vi "Module Loop.vi"(8 "error in (no error)":errorcluster, 11 "Telemetry Server Module in":refnum<class "Telemetry Server Module.lvclass">) -> (0 "error out":errorcluster, 3 "Telemetry Server Module out":refnum<class "Telemetry Server Module.lvclass">)   [LabVIEW 2020, in "Volatus.lvlib" / "Telemetry Server Module.lvclass"]
uses:
  Telemetry Server Module.lvclass
  Telemetry Server Module.lvclass/Telemetry Server Module.ctl
  Module/Module.lvclass
  C:/dev/lv20CE/relink/lv-volatus/Volatus/Module/Module.lvclass
  C:/dev/lv20CE/relink/lv-volatus/Volatus/Telemetry Server Module/Telemetry Server Module.lvclass
  lv-vecto/Vecto/IP Resolver/IP Resolver.lvclass
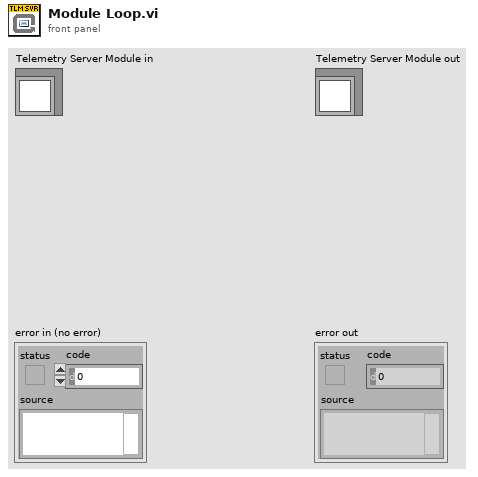
[diagram p1: front panel]
types:
  T1 = enum32{"Invalid", "Standard", "Closed", "Hidden", "Minimized", "Maximized"}
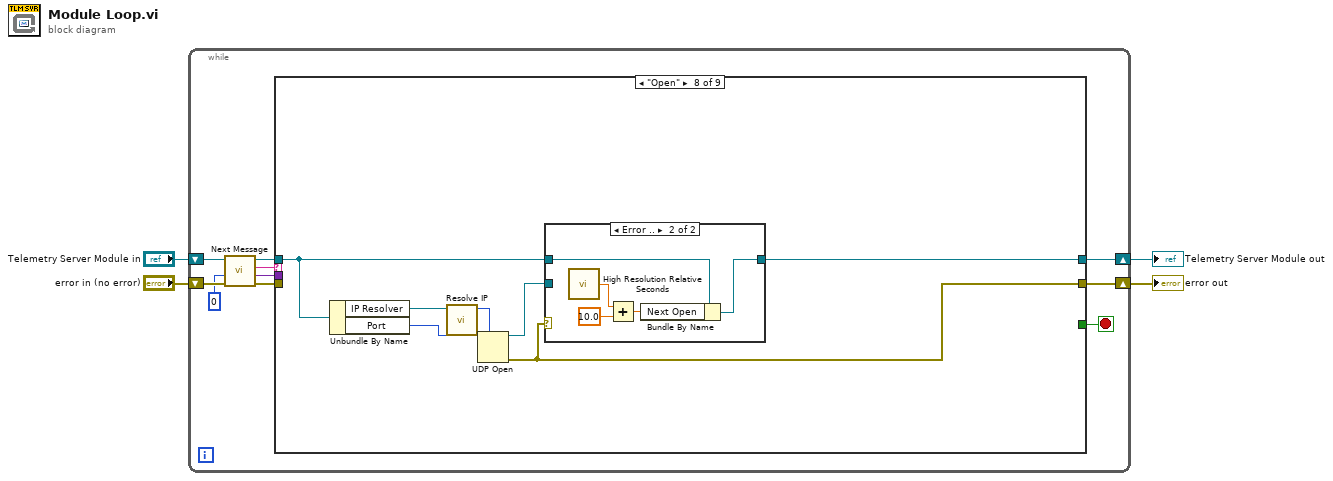
[diagram p0: block diagram]
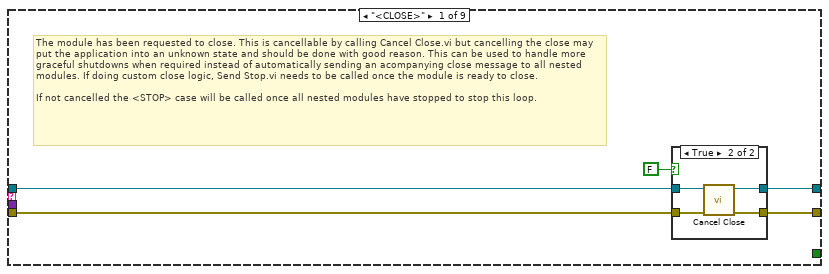
[diagram p2: hidden frame]
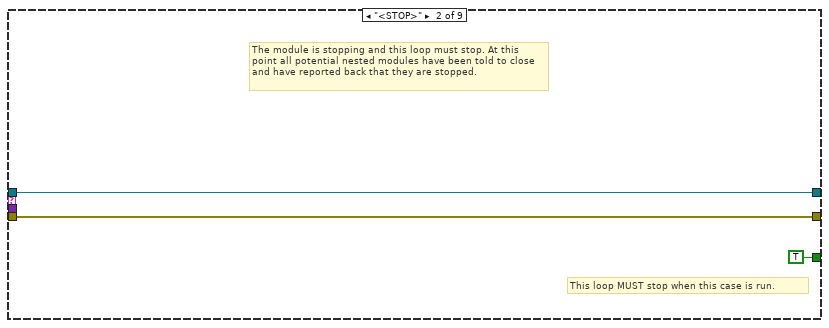
[diagram p4: hidden frame]
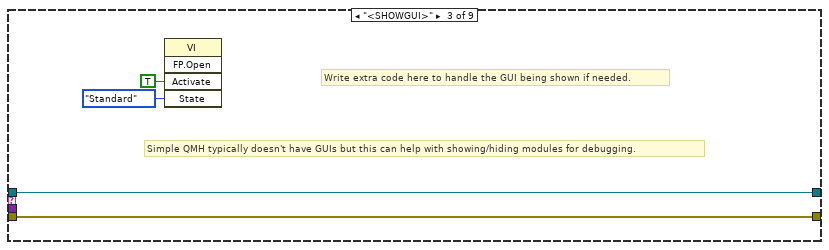
[diagram p5: hidden frame]
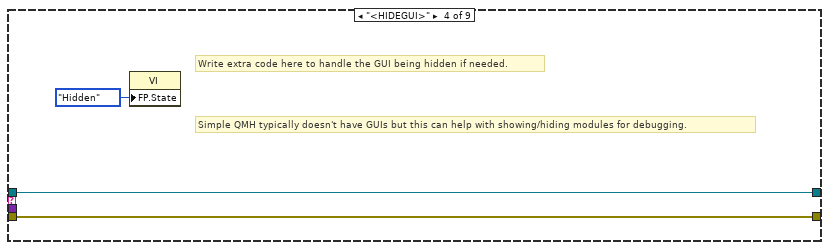
[diagram p6: hidden frame]
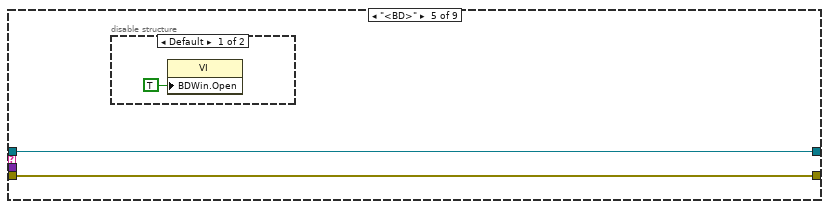
[diagram p7: hidden frame]
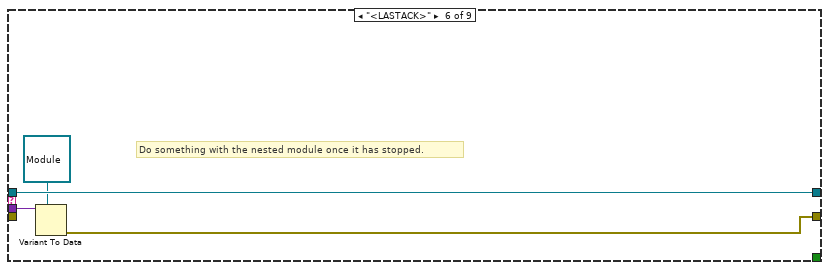
[diagram p9: hidden frame]
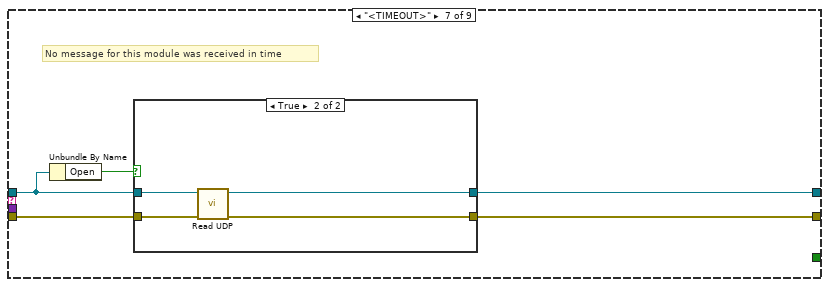
[diagram p10: hidden frame]
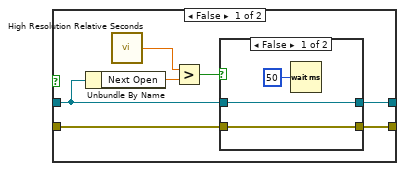
[diagram p11: hidden frame]
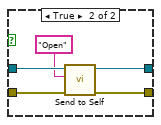
[diagram p12: hidden frame]
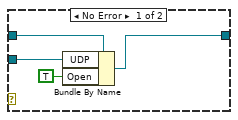
[diagram p13: hidden frame]
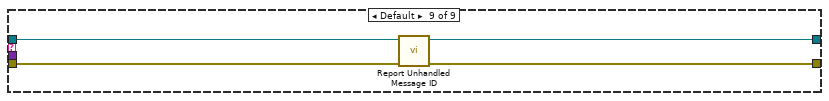
[diagram p14: hidden frame]
diagram:
  n1 = while {
    shift-right: [w9] -> w2
    shift-left: "Telemetry Server Module in" -> [w14]
    shift-right: [w8] -> w1
    shift-left: "error in (no error)" -> [w13]
    stop <- w7 stop-if-true
    n2 = call "Next Message.vi"("error in (no error)"=w13, "Timeout ms (-1)"=0, "Module in"=w14) -> ("error out"=w12:errorcluster, "Data"=w6:variant, "ID"=w11:string, "Module out"=w10:refnum<class "Telemetry Server Module.lvclass">)  [unwired: 5 in]
    n3 = case shown="\"Open\"" w11 {
      tunnel: w12 -> [w19 w27 w31 w34 w36 _ w47 _ w86]
      tunnel: w10 -> [w17 w28 w32 w35 w37 w42 w44 w73 w84]
      tunnel: [w16 w28 w32 w35 w37 w42 w45 w69 w83] -> w9
      tunnel: [w18 w27 w31 w34 w36 w39 w46 w67 w85] -> w8
      tunnel: [_ TRUE _ _ _ _ _ _ _] -> w7
      tunnel: w6 -> [_ _ _ _ _ w41 _ _ _]
      frame "<CLOSE>" {
        # "The module has been requested to close. This is cancellable by calling Cancel Close.vi but cancelling the close may put the application into an unknown state and should be done with good reason. This can be used to handle more graceful shutdowns when required instead of automatically sending an acompanying close message to all nested modules. If doing custom close logic, Send Stop.vi needs to be called once the module is ready to close.\n\nIf not cancelled the <STOP> case will be called once all nested modules have stopped to stop this loop."
        n4 = case shown="True" FALSE {
          tunnel: w19 -> [w20 w25]
          tunnel: [w20 w24] -> w18
          tunnel: w17 -> [w21 w23]
          tunnel: [w21 w22] -> w16
          frame False {
          }
          frame True {
            n5 = call "Cancel Close.vi"("error in (no error)"=w25, "Module in"=w23) -> ("error out"=w24:errorcluster, "Module out"=w22:refnum<class "Telemetry Server Module.lvclass">)  [unwired: 8 in]
          }
        }
      }
      frame "<STOP>" {
        # "This loop MUST stop when this case is run."
        # "The module is stopping and this loop must stop. At this point all potential nested modules have been told to close and have reported back that they are stopped."
      }
      frame "<SHOWGUI>" {
        # "Simple QMH typically doesn't have GUIs but this can help with showing/hiding modules for debugging."
        # "Write extra code here to handle the GUI being shown if needed."
        n6 = invoke class="VI" method="FP.Open"("Activate"=TRUE ("Activate?"), "State"=T1."Standard") -> ()  [unwired: 3 in, 5 out]
      }
      frame "<HIDEGUI>" {
        # "Simple QMH typically doesn't have GUIs but this can help with showing/hiding modules for debugging."
        # "Write extra code here to handle the GUI being hidden if needed."
        n7 = property class="VI"("FP.State"=T1."Hidden" ("Front Panel Window:State")) -> ()  [unwired: 2 in, 2 out]
      }
      frame "<BD>" {
        n8 = disable-structure shown="Default" {
          frame condition #0 (active) {
            n9 = property class="VI"("BDWin.Open"=TRUE ("Block Diagram Window:Open")) -> ()  [unwired: 2 in, 2 out]
          }
          frame condition #1 {
          }
        }
      }
      frame "<LASTACK>" {
        # "Do something with the nested module once it has stopped."
        n10 = Variant To Data(type=refnum<class "Module.lvclass"> refnum ("Volatus:Module"), Variant=w41) -> (error out=w39:errorcluster)  [unwired: 1 in, 1 out]
      }
      frame "<TIMEOUT>" {
        # "No message for this module was received in time"
        n11 = Unbundle By Name(w44) -> ("Open"=w43:bool)
        n12 = case shown="True" w43 {
          tunnel: w47 -> [w51 w66]
          tunnel: [w48 w65] -> w46
          tunnel: [w49 w64] -> w45
          tunnel: w44 -> [w52 w63]
          frame False {
            n13 = Unbundle By Name(w52) -> ("Next Open"=w53:dbl)
            n14 = call <vilib>:"High Resolution Relative Seconds.vi"() -> ("relative seconds"=w54:dbl)
            n15 = Greater?(x=w54, y=w53) -> (0:w50:bool)
            n16 = case shown="False" w50 {
              tunnel: w52 -> [w56 w60]
              tunnel: w51 -> [w55 w62]
              tunnel: [w56 w59] -> w49
              tunnel: [w55 w61] -> w48
              frame False {
                n17 = Wait (ms)(milliseconds to wait=u32 50) -> ()  [unwired: 1 out]
              }
              frame True {
                n18 = call "Send to Self.vi"("error in (no error)"=w62, "Message ID"="Open", "Module in"=w60) -> ("error out"=w61:errorcluster, "Module out"=w59:refnum<class "Telemetry Server Module.lvclass">)  [unwired: 7 in]
              }
            }
          }
          frame True {
            n19 = call "Read UDP.vi"("error in (no error)"=w66, "Telemetry Server Module in"=w63) -> ("error out"=w65:errorcluster, "Telemetry Server Module out"=w64:refnum<class "Telemetry Server Module.lvclass">)  [unwired: 8 in]
          }
        }
      }
      frame "Open" {
        n20 = Unbundle By Name(w73) -> ("IP Resolver"=w72:refnum<class "IP Resolver.lvclass">, "Port"=w70:u16)
        n21 = call "Resolve IP.vi"("IP Resolver in"=w72) -> ("U32 Address"=w71:u32)  [unwired: 9 in, 1 out]
        n22 = UDP Open(7:w71, 11:w70) -> (port=w68:refnum<k16>, 0:w67:errorcluster)  [unwired: 3 in, 1 out]
        n23 = case shown="Error .." w67 {
          tunnel: w73 -> [w77 w82]
          tunnel: [w76 w79] -> w69
          tunnel: w68 -> [w75 _]
          frame No Error {
            n24 = Bundle By Name(cluster=w77, "UDP"=w75, "Open"=TRUE) -> (w76:refnum<class "Telemetry Server Module.lvclass">)
          }
          frame Error {
            n25 = call <vilib>:"High Resolution Relative Seconds.vi"() -> ("relative seconds"=w81:dbl)
            n26 = Add(x=w81, y=10.0) -> (x+y=w78:dbl)
            n27 = Bundle By Name(cluster=w82, "Next Open"=w78) -> (w79:refnum<class "Telemetry Server Module.lvclass">)
          }
        }
      }
      frame Default {
        n28 = call "Report Unhandled Message ID.vi"("error in (no error)"=w86, "Module in"=w84) -> ("error out"=w85:errorcluster, "Module out"=w83:refnum<class "Telemetry Server Module.lvclass">)  [unwired: 8 in]
      }
    }
  }
  "error out" <- w1
  "Telemetry Server Module out" <- w2
